vi "Save Data.vi"(8 "error in":errorcluster, 9 "XY Plot":refnum<vi>, 10 "Plot List":T1(array[cluster]), 11 "DataLog Path":path) -> (0 "error out":errorcluster)   [LabVIEW 2025, in "XY Plotter.lvlib" / "XY Plotter.lvclass"]
uses:
  XY Plotter.lvclass
  <vilib>/Utility/file.llb/Write Delimited Spreadsheet (string).vi
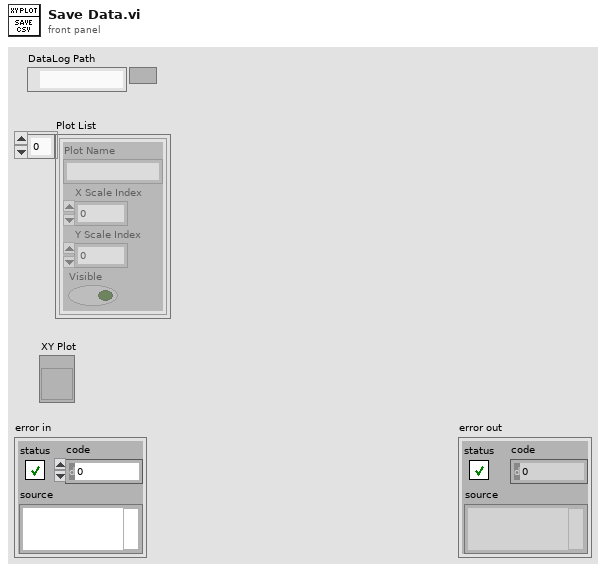
[diagram p1: front panel]
types:
  T1 = cluster{"Plot Name":string, "X Scale Index":u32, "Y Scale Index":u32, "Visible":bool}[]
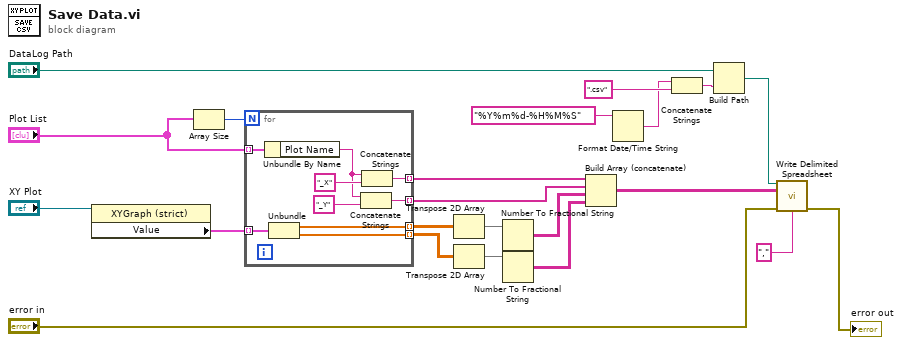
[diagram p0: block diagram]
diagram:
  n1 = property class="XYGraph (strict)"(reference="XY Plot") -> ("Value"=w14:cluster{"Wavenumber":dbl[], "Data":dbl[]}[])  [unwired: 1 in, 2 out]
  n2 = Array Size(array="Plot List") -> (size(s)=w15:i32)
  n3 = for {
    N: w15 -> [_]
    tunnel: w14 -> [w31] mode=indexing
    tunnel: "Plot List" -> [w30] mode=indexing
    tunnel: [w29] -> w13 mode=indexing
    tunnel: [w28] -> w8 mode=indexing
    tunnel: [w24] -> w4 mode=indexing
    tunnel: [w23] -> w3 mode=indexing
    n4 = Unbundle By Name(w30) -> ("Plot Name"=w25:string)
    n5 = Unbundle(w31) -> ("Wavenumber"=w28:dbl[], "Data"=w29:dbl[])
    n6 = Concatenate Strings(w25, "_Y" ("string")) -> (w23:string)
    n7 = Concatenate Strings(w25, "_X" ("string")) -> (w24:string)
  }
  n8 = Transpose 2D Array(2D array=w8) -> (transposed array=w7:dbl[][])
  n9 = Transpose 2D Array(2D array=w13) -> (transposed array=w12:dbl[][])
  n10 = Number To Fractional String(number=w7) -> (F-format string=w5:string[][])  [unwired: 3 in]
  n11 = Number To Fractional String(number=w12) -> (F-format string=w6:string[][])  [unwired: 3 in]
  n12 = Build Array (concatenate)(w4, w3, w5, w6) -> (w16:string[][])
  n13 = Format Date/Time String(time format string (%c)="%Y%m%d-%H%M%S") -> (date/time string=w18:string)  [unwired: 2 in]
  n14 = Concatenate Strings(w18, ".csv" ("string")) -> (w21:string)
  n15 = Build Path(base path="DataLog Path", name or relative path=w21) -> (appended path=w17:path)
  n16 = call-poly <vilib>:"Write Delimited Spreadsheet.vi"("file path (dialog if empty)"=w17, "2D data"=w16, "error in (no error)"="error in", "delimiter (\\t)"="," ("delimiter (\\t)")) -> ("error out"=→"error out":errorcluster)  [unwired: 10 in, 1 out]
